vi "Parse Auto.vi"(11 "Name":string) -> ()   [LabVIEW 2023]
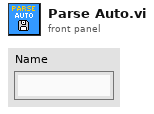
[diagram p1: front panel]
types:
  T1 = typedef "Single Cmd Info.ctl" = cluster{"Name":string, "CPTM.DataType":variant, "All Control Values Variant":cluster{"Name":string, "Variant Data":variant}[], "icon full":T2, "icon scaled":T2, "Path":path, "Subsystem Color":u32}
  T2 = typedef "imagedata.ctl" = cluster{"image type":i32, "image depth":i32, "image":u8[], "mask":u8[], "colors":u32[], "Rectangle":cluster{"left":i16, "top":i16, "right":i16, "bottom":i16}}
  T3 = typedef "Trajectory Data.ctl" = cluster{"Segment Name":string, "Type":T4, "Traj Pos Points":cluster{"x":dbl, "y":dbl, "th":dbl}[], "Traj Vel Points":cluster{"V":dbl, "Omega":dbl, "V vector":cluster{"y":dbl, "x":dbl}}[], "Accel Index":i32, "Decel Index":i32}[]
  T4 = typedef "Segment Type.ctl" = enum16{"Accel Straight", "Const Straight", "Blend", "Circle", "Bezier"}
  T5 = cluster{"Commands out":cluster{"Time (s)":dbl, T1, bool}[], "Zero V":bool, "Trajectory Data":T3, "Reversals":cluster{"Robot Backwards":bool, "Reverse Path":bool}, "Points out":cluster{"x":dbl, "y":dbl, "th":dbl}[]}
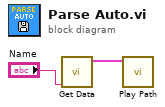
[diagram p0: block diagram]
diagram:
  n1 = call "Get Data.vi"("Name"="Name") -> ("Auto"=w2:T5)  [unwired: 10 in]
  n2 = call "Play Path.vi"("Auto Data"=w2) -> ()  [unwired: 10 in, 1 out]
